vi "uService GUI.vi"(8 "error in (no error)":errorcluster, 11 "Monkey in":refnum<class "Monkey.lvclass">) -> (3 "Monkey out":refnum<class "Monkey.lvclass">)   [LabVIEW 2020, in "Monkey.lvlib" / "Monkey.lvclass"]
uses:
  Monkey.lvclass
  C:/LabVIEW Code/CIRCUS/TALOS/TALOS_PPL.lvlibp/Father of all uServices/Father of all uServices/Father of all uServices.lvclass
  Run Utilities/Schedule/Array of Runs - GUI.ctl
  Run Utilities/Cell/Cell - GUI.ctl
  Run Utilities/Run Instance/Run Instance - GUI.ctl
  Monkey Consumer Case Selector.ctl
  fd9ba2b9-9de8-4540-b686-759542742d7d.vi
  fd9ba2b9-9de8-4540-b686-759542742d7d.vi/d4db2432-cc9c-482c-8957-dac855435ef6.vi
  fd9ba2b9-9de8-4540-b686-759542742d7d.vi/86fbf154-bd7b-49a2-8ab2-a837b2a95f24.vi
  fd9ba2b9-9de8-4540-b686-759542742d7d.vi/3b95b01e-1ec2-4565-bcd9-7606a5281010.vi
  fd9ba2b9-9de8-4540-b686-759542742d7d.vi/96a08935-737a-44b2-979c-a81d56408f7e.vi
  fd9ba2b9-9de8-4540-b686-759542742d7d.vi/d4db2432-cc9c-482c-8957-dac855435ef6.vi/6eaecd13-6e48-4772-a921-b51ebdf84d88.vi
  fd9ba2b9-9de8-4540-b686-759542742d7d.vi/d4db2432-cc9c-482c-8957-dac855435ef6.vi/d2d5f2b7-06f4-47f6-971c-049c3fdbb653.vi
  fd9ba2b9-9de8-4540-b686-759542742d7d.vi/3b95b01e-1ec2-4565-bcd9-7606a5281010.vi/6eaecd13-6e48-4772-a921-b51ebdf84d88.vi
  fd9ba2b9-9de8-4540-b686-759542742d7d.vi/3b95b01e-1ec2-4565-bcd9-7606a5281010.vi/d2d5f2b7-06f4-47f6-971c-049c3fdbb653.vi
  fd9ba2b9-9de8-4540-b686-759542742d7d.vi/96a08935-737a-44b2-979c-a81d56408f7e.vi/6eaecd13-6e48-4772-a921-b51ebdf84d88.vi
  fd9ba2b9-9de8-4540-b686-759542742d7d.vi/96a08935-737a-44b2-979c-a81d56408f7e.vi/d2d5f2b7-06f4-47f6-971c-049c3fdbb653.vi
  <vilib>/Comparison/Less/Less Functor/Less Functor.lvclass
  TALOS/TALOS_PPL.lvlibp/Father of all uServices/Father of all uServices/Father of all uServices.lvclass
  Run Utilities/Run Instance/Run Instance.lvclass
  Run Utilities/Schedule/Schedule.lvclass
  Run Utilities/Cell/Schedule Cell.lvclass
panel:
  in  "Delete cell":bool
  in  "Move down":bool
  in  "Move up":bool
  in  "Cell index":i32=-1
  in  "Skip schedule":bool
  out "Stopped":bool
  out "Paused":bool
  in  "Monkey Picture":picture
  out "Error Criticality":u8 max=4
  out "uS ID":string
  out "Synchronised":bool
  out "Continuous":bool
  out "Current RUN":T1
  out "ETA":string
  out "Scripts left":dbl
  out "Skipped RUNs":T2 {"Number of cycles" min=1}
  out "Report from previous RUNs":string
  out "Current Action":string
  out "RUNs Schedule":T2 {"Number of cycles" min=1}
  in  "stop Monkey":bool
  # "Run Information"
  # "Schedule manipulation"
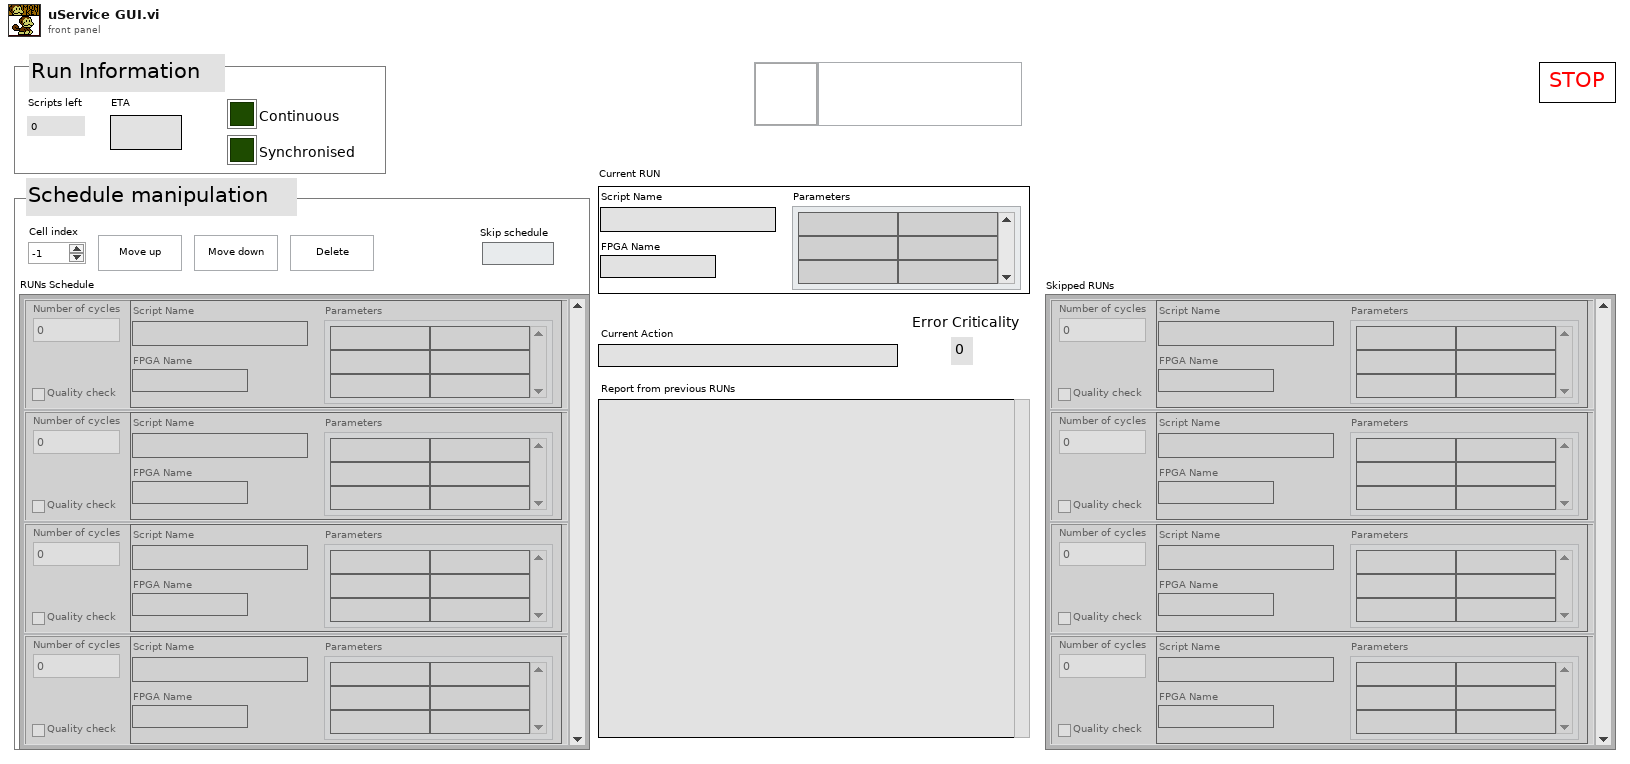
[diagram p1: front panel]
types:
  T1 = typedef "Run Utilities.lvlib/Run Instance.lvclass/Run Instance - GUI.ctl" = cluster{"Script Name":string, "Parameters":string[][], "FPGA Name":string}
  T2 = typedef "Run Utilities.lvlib/Schedule.lvclass/Array of Runs - GUI.ctl" = T3[]
  T3 = typedef "Run Utilities.lvlib/Schedule Cell.lvclass/Cell - GUI.ctl" = cluster{"Background Color":u32, "Number of cycles":u32, "Single RUN":T1, "Quality check":bool, "Cell Type":string}
  T4 = typedef "Monkey.lvlib/Monkey.lvclass/Monkey Consumer Case Selector.ctl" = enum16{"Init", "Update GUI", "New schedule", "Check Script", "Submit Script", "Banana arrived", "Optimiser - evaluate RUN", "Optimiser - update RUN", "Quality Check", "What to do next", "Update Crit Lvl", "Skip Run", "Stop Schedule", "Skip schedule", "Append", "Update index", "Delete cell", "Move cell"}
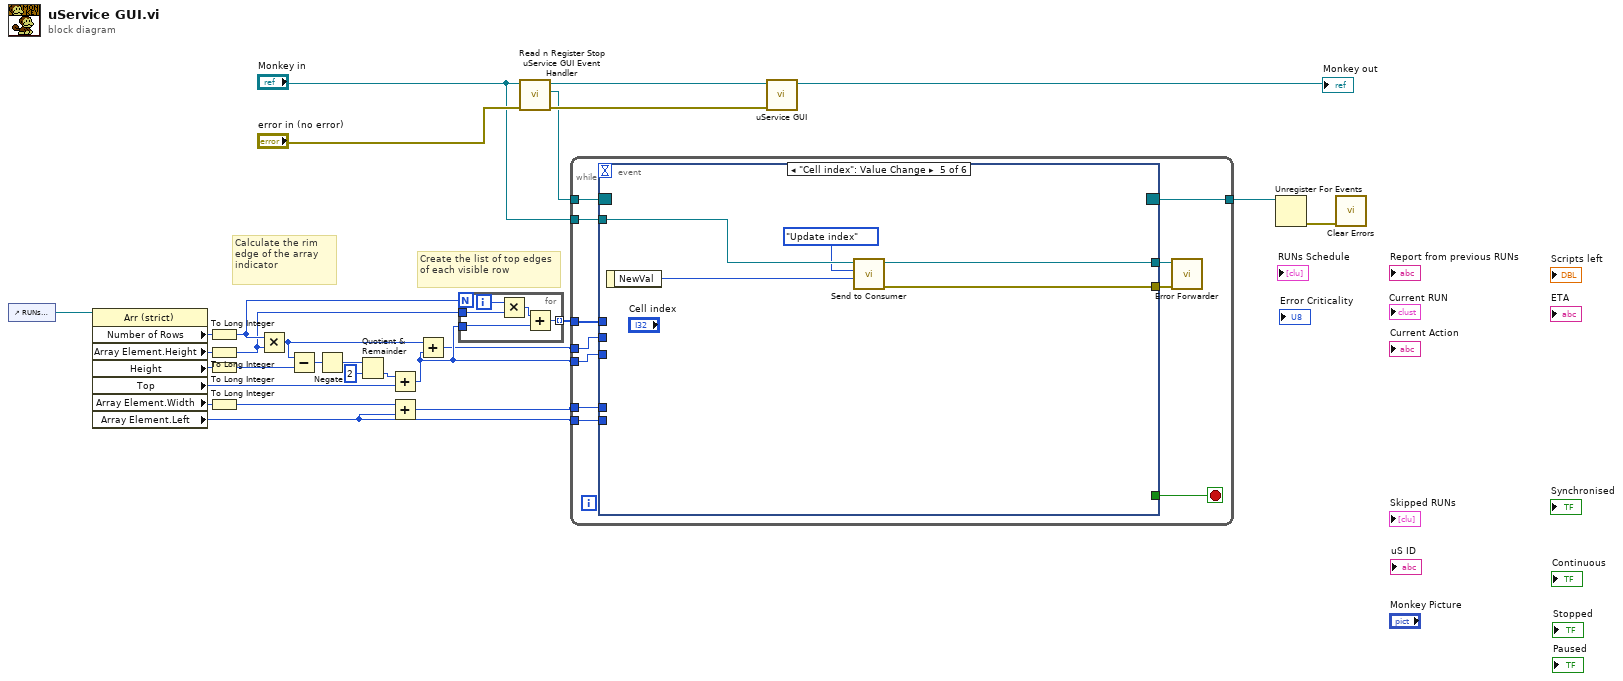
[diagram p0: block diagram]
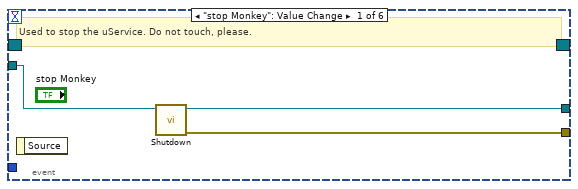
[diagram p2: hidden frame]
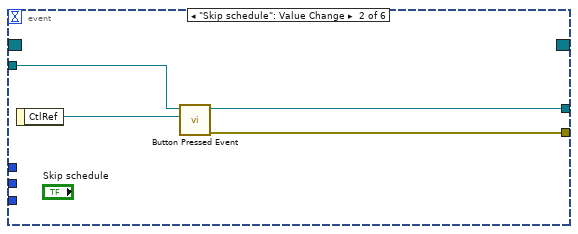
[diagram p3: hidden frame]
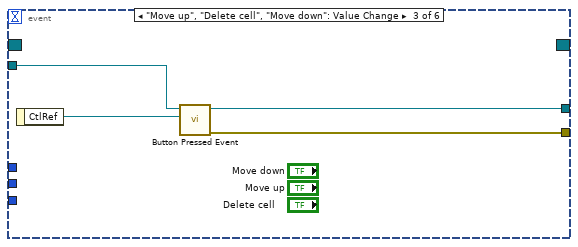
[diagram p4: hidden frame]
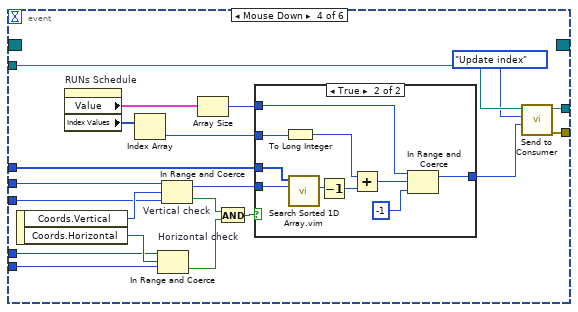
[diagram p5: hidden frame]
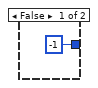
[diagram p6: hidden frame]
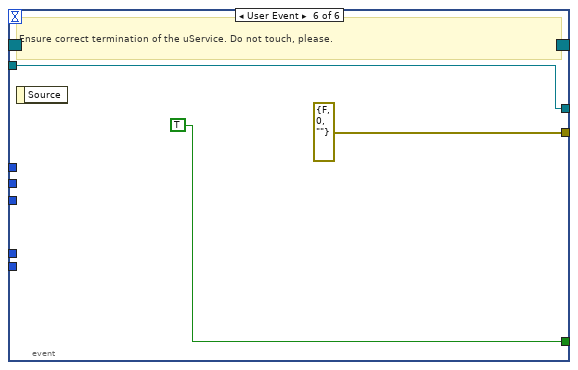
[diagram p7: hidden frame]
diagram:
  # "Create the list of top edges of each visible row"
  # "Calculate the rim edge of the array indicator"
  n1 = control-ref of="RUNs Schedule"() -> (w6:refnum<vi>)
  n2 = property class="Arr (strict)"(reference=w6) -> ("Number of Rows"=w14:u32, "Array Element.Height"=w12:u32, "Height"=w16:u32, "Top"=w9:i32, "Array Element.Width"=w18:u32, "Array Element.Left"=w5:i32)  [unwired: 1 in, 2 out]
  n3 = To Long Integer(number=w14) -> (32bit integer=w13:i32)
  n4 = To Long Integer(number=w12) -> (32bit integer=w11:i32)
  n5 = To Long Integer(number=w16) -> (32bit integer=w15:i32)
  n6 = To Long Integer(number=w18) -> (32bit integer=w19:i32)
  n7 = Multiply(x=w13, y=w11) -> (x*y=w8:i32)
  n8 = Subtract(x=w8, y=w15) -> (x-y=w10:i32)
  n9 = Negate(x=w10) -> (-x=w7:i32)
  n10 = Quotient & Remainder(x=w7, y=2) -> (floor(x/y)=w17:i32)  [unwired: 1 out]
  n11 = Add(x=w17, y=w9) -> (x+y=w3:i32)
  n12 = Add(x=w19, y=w5) -> (x+y=w4:i32)
  n13 = Add(x=w8, y=w3) -> (x+y=w2:i32)
  n14 = for {
    N: w13 -> [_]
    tunnel: [w33] -> w1 mode=indexing
    tunnel: w11 -> [w31]
    tunnel: w3 -> [w29]
    i -> [w30]
    n15 = Multiply(x=w30, y=w31) -> (x*y=w32:i32)
    n16 = Add(x=w32, y=w29) -> (x+y=w33:i32)
  }
  n17 = call-dynamic "Read n Register Stop uService GUI Event Handler .vi"("error in (no error)"="error in (no error)", "uService Template in"="Monkey in") -> ("error out"=w26:errorcluster, "Stop uService GUI Event Ref"=w25:refnum<event-registration>, "uService Template out"=w27:refnum<class "Monkey.lvclass">)  [unwired: 7 in]
  n18 = while {
    tunnel: [w44] -> w28
    tunnel: w25 -> [w42]
    tunnel: "Monkey in" -> [w41]
    tunnel: w2 -> [w35]
    tunnel: w3 -> [w36]
    tunnel: w5 -> [w37]
    tunnel: w4 -> [w38]
    tunnel: w1 -> [w34]
    stop <- w43 stop-if-true
    n19 = event shown="[4] \"Cell index\": Value Change" {
      selector: w42 -> [_ _ _ _ _ _]
      dyn-events: [_ _ _ _ _ _] -> w44
      timeout: _ -> [_ _ _ _ _ _]
      tunnel: [_ _ _ _ _ TRUE] -> w43
      tunnel: w41 -> [w47 w51 w55 w75 w91 w93]
      tunnel: [w46 w49 w53 w57 w89 w93] -> w40
      tunnel: [w45 w48 w52 w58 w88 errorcluster {"status"=FALSE, "code"=0, "source"=""} ("error out")] -> w39
      tunnel: w38 -> [_ _ _ w73 _ _]
      tunnel: w37 -> [_ _ _ w72 _ _]
      tunnel: w36 -> [_ _ _ w70 _ _]
      tunnel: w35 -> [_ _ _ w69 _ _]
      tunnel: w34 -> [_ _ _ w61 _ _]
      event "stop Monkey": Value Change {
        # "Used to stop the uService. Do not touch, please."
        n20 = event-data() -> ()  [unwired: 1 in, 1 out]
        n21 = call "Shutdown.vi"("Father of all uServices in"=w47) -> ("error out"=w45:errorcluster, "Father of all uServices out"=w46:refnum<class "Monkey.lvclass">)  [unwired: 9 in]
      }
      event "Skip schedule": Value Change {
        n22 = event-data() -> ("CtlRef"=w50:refnum<vi>)  [unwired: 1 in]
        n23 = call-dynamic "Button Pressed Event.vi"("CtlRef"=w50, "uService Template in"=w51) -> ("error out"=w48:errorcluster, "uService Template out"=w49:refnum<class "Monkey.lvclass">)  [unwired: 8 in]
      }
      event "Move up", "Delete cell", "Move down": Value Change {
        n24 = event-data() -> ("CtlRef"=w54:refnum<vi>)  [unwired: 1 in]
        n25 = call-dynamic "Button Pressed Event.vi"("CtlRef"=w54, "uService Template in"=w55) -> ("error out"=w52:errorcluster, "uService Template out"=w53:refnum<class "Monkey.lvclass">)  [unwired: 8 in]
      }
      event Mouse Down {
        n26 = event-data() -> ("Coords.Vertical"=w71:i32, "Coords.Horizontal"=w74:i32)  [unwired: 1 in]
        n27 = property on="RUNs Schedule" class="Arr (strict)"() -> ("Value"=w68:T2, "Index Values"=w66:u32[])  [unwired: 2 in, 2 out]
        n28 = Index Array(array=w66) -> (element=w65:u32)  [unwired: 1 in]
        n29 = In Range and Coerce "Horizontal check"(upper limit=w73, x=w74, lower limit=w72) -> (In Range?=w62:bool)  [unwired: 1 out]
        n30 = In Range and Coerce "Vertical check"(upper limit=w69, x=w71, lower limit=w70) -> (coerced(x)=w60:i32, In Range?=w63:bool)
        n31 = Array Size(array=w68) -> (size(s)=w67:i32)
        n32 = And(x=w63, y=w62) -> (x .and. y?=w64:bool)
        n33 = case shown="True" w64 {
          tunnel: w67 -> [_ w80]
          tunnel: w65 -> [_ w82]
          tunnel: w61 -> [_ w86]
          tunnel: w60 -> [_ w85]
          tunnel: [-1 ("t") w77] -> w56
          frame False {
          }
          frame True {
            n34 = To Long Integer(number=w82) -> (32bit integer=w81:i32)
            n35 = call "Search Sorted 1D Array.vim"("element"=w85, "sorted 1D array"=w86) -> ("nearest index"=w84:i32)  [unwired: 8 in, 1 out]
            n36 = Decrement(x=w84) -> (x-1=w83:i32)
            n37 = Add(x=w81, y=w83) -> (x+y=w78:i32)
            n38 = In Range and Coerce(upper limit=w80, x=w78, lower limit=-1) -> (coerced(x)=w77:i32)  [unwired: 1 out]
          }
        }
        n39 = call "Send to Consumer.vi"("Data"=w56, "Case ID"=Monkey_Consumer_Case_Selector."Update index" ("Monkey Consumer Case Selector"), "uService Template in"=w75) -> ("error out"=w58:errorcluster, "uService Template out"=w57:refnum<class "Monkey.lvclass">)  [unwired: 7 in]
      }
      event "Cell index": Value Change {
        n40 = event-data() -> ("NewVal"=w87:i32)  [unwired: 1 in]
        n41 = call "Send to Consumer.vi"("Data"=w87, "Case ID"=Monkey_Consumer_Case_Selector."Update index" ("Monkey Consumer Case Selector"), "uService Template in"=w91) -> ("error out"=w88:errorcluster, "uService Template out"=w89:refnum<class "Monkey.lvclass">)  [unwired: 7 in]
      }
      event User Event {
        # "Ensure correct termination of the uService. Do not touch, please."
        n42 = event-data() -> ()  [unwired: 1 in, 1 out]
      }
    }
    n43 = call "Error Forwarder.vi"("error in (no error)"=w39, "Father of all uServices in"=w40) -> ()  [unwired: 10 in]
  }
  n44 = call-parent "uService GUI.vi"("error in (no error)"=w26, "uService Template in"=w27) -> ("uService Template out"=→"Monkey out":refnum<class "Monkey.lvclass">)  [unwired: 9 in]
  n45 = Unregister For Events(event registration refnum=w28) -> (error out=w21:errorcluster)  [unwired: 1 in]
  n46 = call <vilib>:"Clear Errors.vi"("error in (no error)"=w21) -> ()  [unwired: 5 in, 2 out]
